vi "Get Tests Events by Key.vi"(8 "error in (no error)":errorcluster, 10 "Key (Test ID)":string, 11 "Test Event Storage in":refnum<class "Test Event Storage.lvclass">) -> (0 "error out":errorcluster, 1 "Assertions":T1[](array[typedef]), 3 "Test Event Storage out":refnum<class "Test Event Storage.lvclass">)   [LabVIEW 2020, in "Caraya.lvlib" / "Test Event Storage.lvclass"]
uses:
  Test Event Storage.lvclass
  Test Result/Assert Event Data (Extended).ctl
  test store -- cluster.ctl
  Test Manager Message Test/TestManagerMsg.Test.lvclass
  assert store -- cluster.ctl
  Test Manager Message Assertion/TestManagerMsg.Assertion.lvclass
  Test Manager Message Verbose/TestManagerMsg.Verbose.lvclass
  Test Event Storage.lvclass/Test Event Storage.ctl
  Test Result/Test Result.lvclass
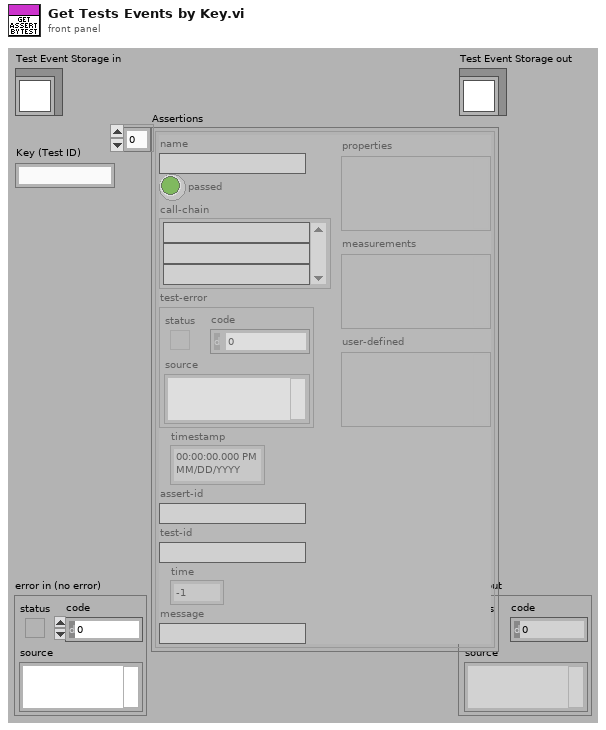
[diagram p1: front panel]
types:
  T1 = typedef "Caraya.lvlib/Test Result.lvclass/Assert Event Data (Extended).ctl" = cluster{"name":string, "passed":bool, "call-chain":string[], "test-error":errorcluster, "timestamp":timestamp, "assert-id":string, "test-id":string, "time":dbl, "message":string, "properties":variant, "measurements":variant, "user-defined":variant}
  T2 = typedef "Caraya.lvlib/Test Event Storage.lvclass/assert store -- cluster.ctl" = cluster{"Assertion":refnum<class "TestManagerMsg.Assertion.lvclass">, "Explanation":refnum<class "TestManagerMsg.Verbose.lvclass">, "properties":variant, "measurements":variant, "user-defined":variant}
  T3 = typedef "Caraya.lvlib/Test Event Storage.lvclass/test store -- cluster.ctl" = cluster{"Test":refnum<class "TestManagerMsg.Test.lvclass">, "Defined":bool, "Passed":bool, "properties":variant, "assert-ids":variant}
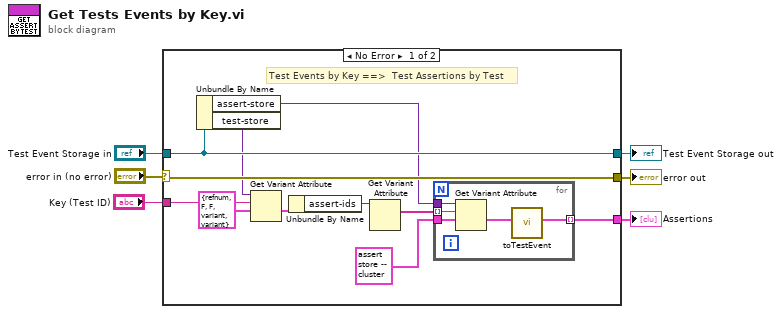
[diagram p0: block diagram]
diagram:
  n1 = case shown="No Error" "error in (no error)" {
    selector: "error in (no error)" -> [w16 w24]
    tunnel: [w16 w24] -> w5
    tunnel: [w14 w23] -> w3
    tunnel: "Test Event Storage in" -> [w14 w23]
    tunnel: "Key (Test ID)" -> [w17 _]
    tunnel: [w15 _] -> w1
    frame No Error {
      # "Test Events by Key ==>  Test Assertions by Test"
      n2 = Unbundle By Name(w14) -> ("assert-store"=w11:variant, "test-store"=w13:variant)
      n3 = Get Variant Attribute(Variant=w13, name=w17, default value (empty Variant)=T3 {"Test"=refnum, "Defined"=FALSE, "Passed"=FALSE, "properties"=variant, "assert-ids"=variant} ("test-store")) -> (value=w9:T3)  [unwired: 1 in, 3 out]
      n4 = Unbundle By Name(w9) -> ("assert-ids"=w8:variant)
      n5 = Get Variant Attribute(Variant=w8) -> (names=w7:string[])  [unwired: 3 in, 3 out]
      n6 = for {
        tunnel: w11 -> [w22]
        tunnel: w7 -> [w21] mode=indexing
        tunnel: T2 {"Assertion"=refnum, "Explanation"=refnum, "properties"=variant, "measurements"=variant, "user-defined"=variant} ("assert-store") -> [w20]
        tunnel: [w18] -> w15 mode=indexing
        n7 = Get Variant Attribute(Variant=w22, name=w21, default value (empty Variant)=w20) -> (value=w19:T2)  [unwired: 1 in, 3 out]
        n8 = call "toTestEvent.vi"("assert-store"=w19) -> ("Assert Event Data"=w18:T1)  [unwired: 10 in]
      }
    }
    frame Error {
    }
  }
  "error out" <- w5
  "Test Event Storage out" <- w3
  "Assertions" <- w1
